vi "RemoteVI Restore If Minimized.vi"(0 "hWnd":u64, 11 "error in":errorcluster) -> (4 "was minimized?":bool, 15 "error out":errorcluster)   [LabVIEW 2020, in "RemoteVI.lvlib"]
doc: "Restores the window hWnd when it is minimized - a minimized front panel ignores posted input - with ShowWindow(hWnd, 4 SW_SHOWNOACTIVATE), which brings it back WITHOUT activating it or taking the focus. A window that is not minimized is left alone. Win32 calls only (IsIconic, ShowWindow), no VI Server, so it also works while LabVIEW's UI thread is blocked."
uses:
  RemoteVI.lvlib
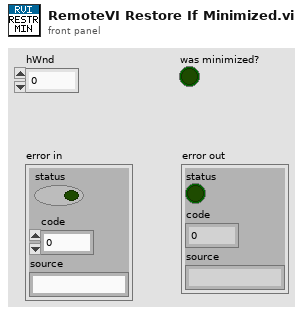
[diagram p1: front panel]
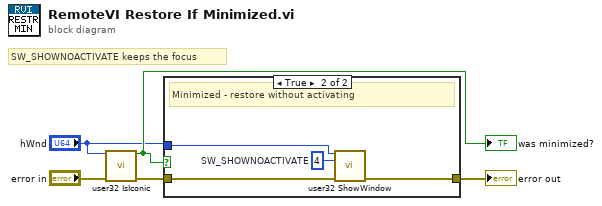
[diagram p0: block diagram]
diagram:
  # "SW_SHOWNOACTIVATE keeps the focus"
  n1 = call "user32 IsIconic.vi"("hWnd"="hWnd", "error in"="error in") -> ("minimized?"=w3:bool, "error out"=w5:errorcluster)  [unwired: 12 in]
  "was minimized?" <- w3
  n2 = case shown="True" w3 {
    tunnel: "hWnd" -> [_ w7]
    tunnel: w5 -> [w6 w8]
    tunnel: [w6 w10] -> w4
    frame False {
      # "Not minimized - nothing to do"
    }
    frame True {
      w9 = 4  # SW_SHOWNOACTIVATE
      # "Minimized - restore without activating"
      n3 = call "user32 ShowWindow.vi"("hWnd"=w7, "nCmdShow"=w9, "error in"=w8) -> ("error out"=w10:errorcluster)  [unwired: 11 in, 1 out]
    }
  }
  "error out" <- w4
